vi "update VISA Resource.vi"(8 "error in (no error)":errorcluster, 10 "VISA resource name":refnum<visa-resource-name>, 11 "FSV-40N in":refnum<class "FSV-40N.lvclass">) -> (0 "error out":errorcluster, 3 "FSV-40N out":refnum<class "FSV-40N.lvclass">)   [LabVIEW 2023, in "Spectrum Analyzer.lvlib" / "FSV-40N.lvclass"]
uses:
  FSV-40N.lvclass
  FSV-40N.lvclass/FSV-40N.ctl
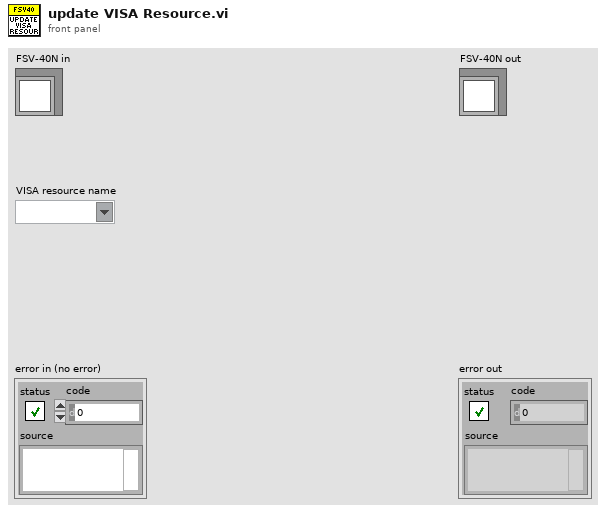
[diagram p1: front panel]
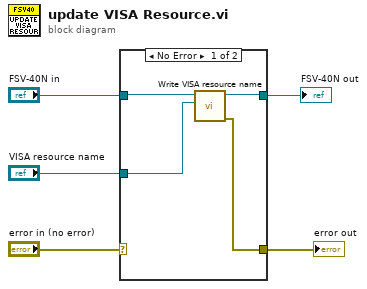
[diagram p0: block diagram]
diagram:
  n1 = case shown="No Error" "error in (no error)" {
    selector: "error in (no error)" -> [_ w11]
    tunnel: "FSV-40N in" -> [w9 w10]
    tunnel: [w7 w11] -> w3
    tunnel: [w6 w10] -> w2
    tunnel: "VISA resource name" -> [w8 _]
    frame No Error {
      n2 = call "Write VISA resource name.vi"("VISA resource name"=w8, "FSV-40N in"=w9) -> ("error out"=w7:errorcluster, "FSV-40N out"=w6:refnum<class "FSV-40N.lvclass">)  [unwired: 8 in]
    }
    frame Error {
    }
  }
  "error out" <- w3
  "FSV-40N out" <- w2
